vi "hmb!.vi"() -> ()   [LabVIEW 2023]
panel:
  out "Waveform Graph":dbl[](graph)
  in  "measurements\n(AC level) 3":u16(ring) items=["AC level", "DC level", "Distortion", "Distortion level", "Signal-to-Noise", "SINAD"]
  in  "error in (no error) 4":errorcluster
  out "Y vs. Frequency":cluster{dbl, dbl}[](graph)
  in  "error in (no error) 3":errorcluster
  in  "measurements\n(AC level) 2":u16(ring) items=["AC level", "DC level", "Distortion", "Distortion level", "Signal-to-Noise", "SINAD"]
  in  "stop frequency (Hz)":dbl=30000.0 min=20.0 max=100000.0 format="%.5f"
  in  "start frequency (Hz)":dbl=50.0 min=20.0 max=100000.0 format="%.5f"
  in  "sweep resolution\n(5points/decade)":u16(ring)=2 items=["1 point/decade", "2 points/decade", "5 points/decade", "10 points/decade", "20 points/decade", "50 points/decade", "100 points/decade", "200 points/decade", "500 points/decade"]
  out "value read":dbl format="%.7f"
  in  "measurements\n(AC level)":u16(ring) items=["AC level", "DC level", "Distortion", "Distortion level", "Signal-to-Noise", "SINAD"]
  in  "detector selection\n(no change)":u16(ring) items=["no change", "rms", "average", "quasi-peak"]
  in  "error in (no error) 2":errorcluster
  out "VISA session":refnum<visa-resource-name>
  out "error out":errorcluster
  in  "VISA resource name":refnum<visa-resource-name>
  in  "reset (no : F)":bool
  in  "error in (no error)":errorcluster
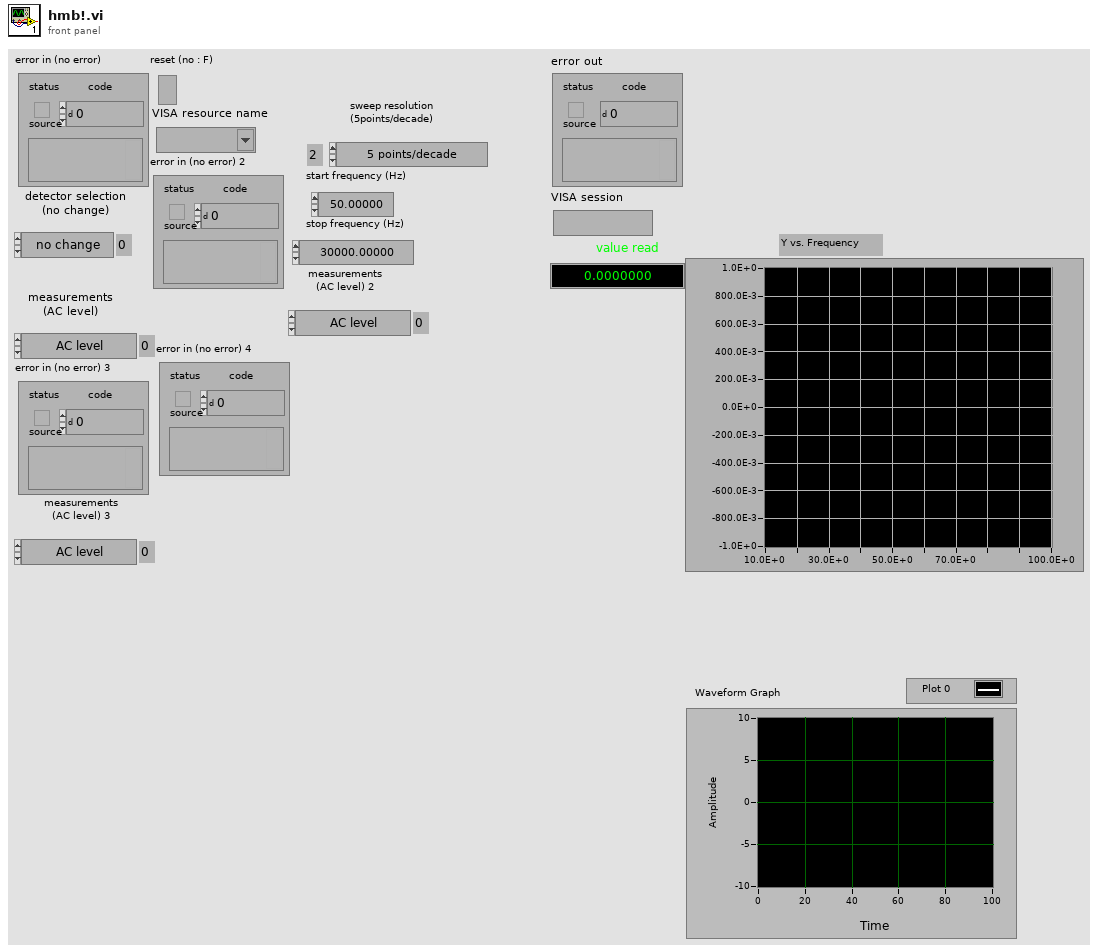
[diagram p1: front panel]
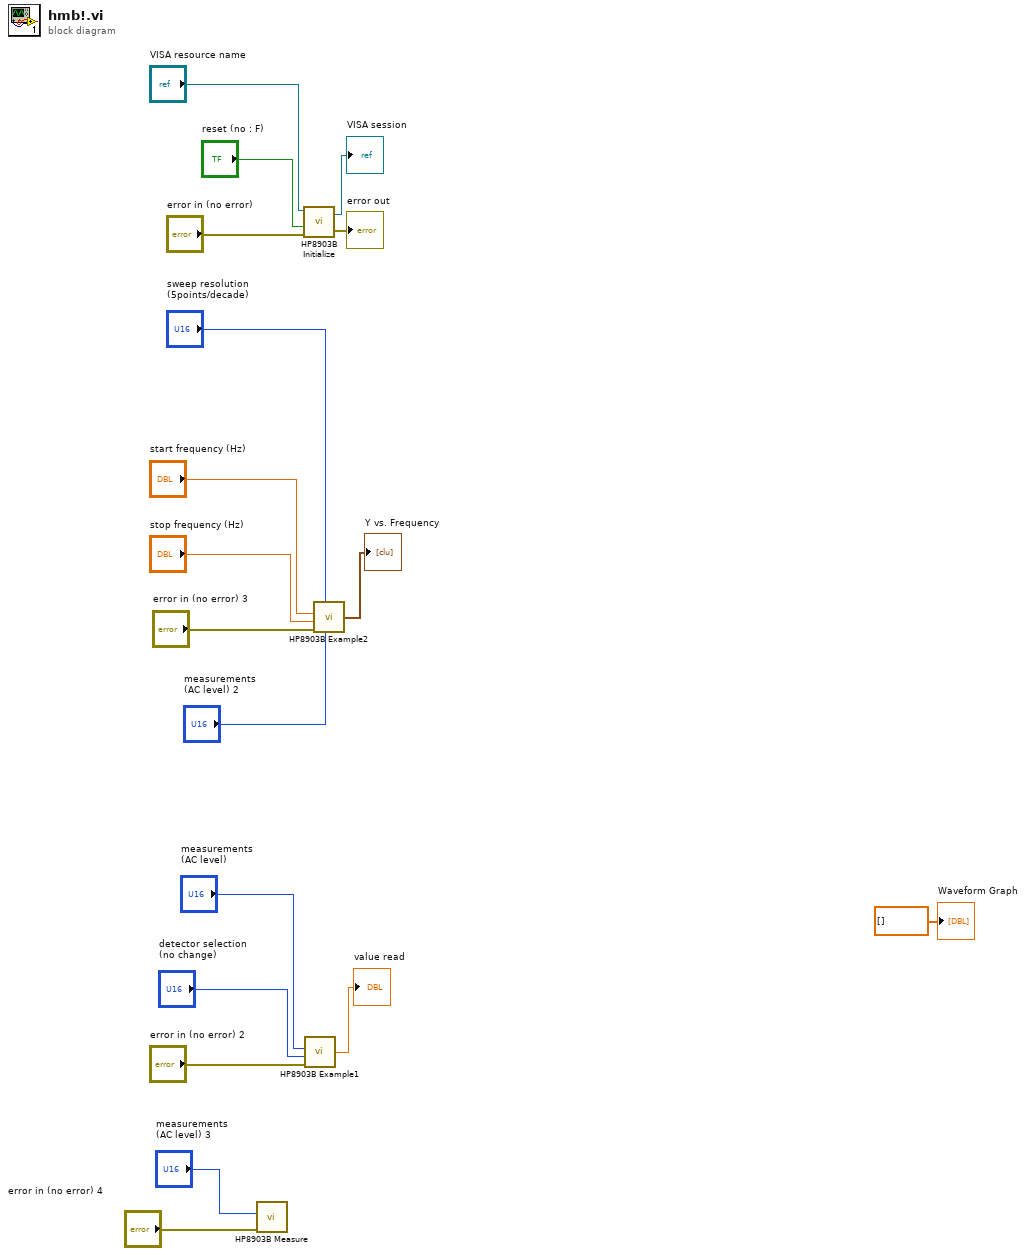
[diagram p0: block diagram]
diagram:
  n1 = call <instrlib>:"HP8903B Measure.vi"("error in (no error)"="error in (no error) 4", "measurements\n(AC level)"="measurements\n(AC level) 3") -> ()  [unwired: 2 in, 3 out]
  n2 = call <instrlib>:"HP8903B Initialize.vi"("error in (no error)"="error in (no error)", "reset (no : F)"="reset (no : F)", "VISA resource name"="VISA resource name") -> ("error out"=→"error out":errorcluster, "VISA session"=→"VISA session":refnum<visa-resource-name>)  [unwired: 1 in]
  n3 = call <instrlib>:"HP8903B Example1.vi"("error in (no error)"="error in (no error) 2", "detector selection\n(no change)"="detector selection\n(no change)", "measurements\n(AC level)"="measurements\n(AC level)") -> ("value read"=→"value read":dbl)  [unwired: 1 in, 2 out]
  n4 = call <instrlib>:"HP8903B Example2.vi"("sweep resolution\n(5points/decade)"="sweep resolution\n(5points/decade)", "start frequency (Hz)"="start frequency (Hz)", "stop frequency (Hz)"="stop frequency (Hz)", "measurements\n(AC level)"="measurements\n(AC level) 2", "error in (no error)"="error in (no error) 3") -> ("Y vs. Frequency"=→"Y vs. Frequency":cluster{dbl, dbl}[])  [unwired: 1 in, 2 out]
  "Waveform Graph" <- dbl[] [] ("Waveform Graph")
